vi "shear_and_recovery_calculation__0b88896683.vi"(6 "stop steps":i32, 8 "loop period (ms)":dbl, 9 "# periods":dbl, 10 "recovery phase":dbl, 11 "frequency":dbl) -> (1 "Time needed":dbl, 2 "shear+stop points":dbl, 3 "shear points":dbl)   [LabVIEW 2023]
uses:
  <vilib>/Analysis/NI_AALBase.lvlib
panel:
  out "element":dbl
  in  "amplitude":dbl=1.0 format="%0.2f"
  out "recovery phase points":dbl
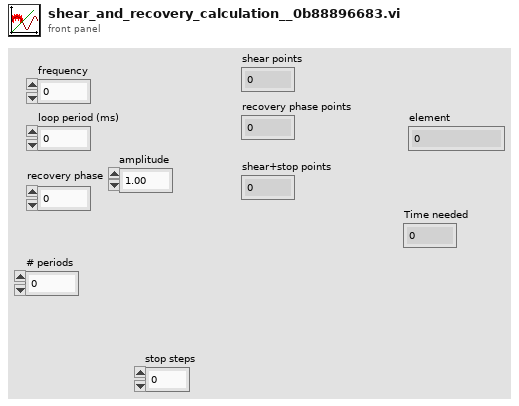
[diagram p1: front panel]
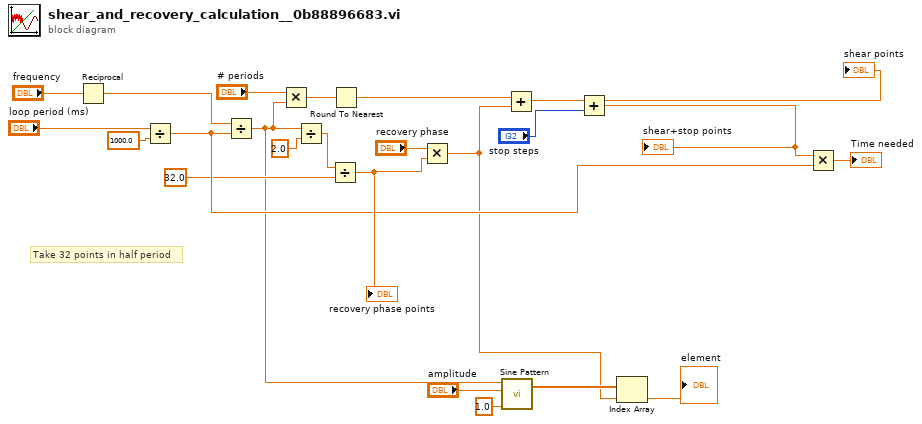
[diagram p0: block diagram]
diagram:
  # "Take 32 points in half period"
  n1 = Reciprocal(x="frequency") -> (1/x=w20:dbl)
  n2 = Divide(x="loop period (ms)", y=1000.0) -> (x/y=w11:dbl)
  n3 = Divide(x=w20, y=w11) -> (x/y=w5:dbl)
  n4 = Multiply(x="# periods", y=w5) -> (x*y=w23:dbl)
  n5 = Divide(x=w5, y=2.0) -> (x/y=w15:dbl)
  n6 = Divide(x=w15, y=32.0) -> (x/y=w14:dbl)
  "recovery phase points" <- w14
  n7 = Round To Nearest(number=w23) -> (nearest integer value=w13:dbl)
  n8 = Multiply(x="recovery phase", y=w14) -> (x*y=w1:dbl)
  n9 = call <vilib>:"Sine Pattern.vi"("cycles"=1.0, "amplitude"="amplitude", "samples"=w5) -> ("Sinusoidal Pattern"=w3:dbl[])  [unwired: 1 in, 1 out]
  n10 = Add(x=w13, y=w1) -> (x+y=w9:dbl)
  "shear points" <- w9
  n11 = Add(x=w9, y="stop steps") -> (x+y=w12:dbl)
  "shear+stop points" <- w12
  n12 = Index Array(array=w3, index=w1) -> (element=→"element":dbl)
  n13 = Multiply(x=w12, y=w11) -> (x*y=→"Time needed":dbl)
